vi "Double Array.vi"(8 "Error In":errorcluster) -> (0 "Error Out":errorcluster)   [LabVIEW 2018, in "Tests.lvlib" / "To Msgpack.lvlib"]
uses:
  To Msgpack.lvlib
  <vilib>/addons/_JKI Toolkits/Caraya/classes/Test/Test.lvclass
  src/Toolkit/Toolkit.lvlib
  <vilib>/addons/_JKI Toolkits/Caraya/classes/Assert/Assert.lvclass
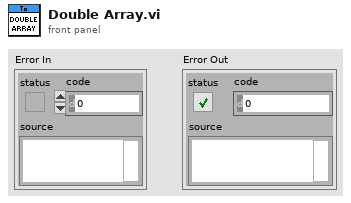
[diagram p1: front panel]
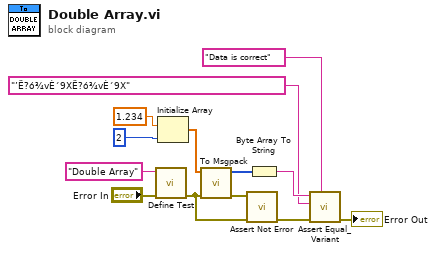
[diagram p0: block diagram]
diagram:
  n1 = call <vilib>:"Define Test.vi"("error in (no error)"="Error In", "Label (VI Title)"="Double Array") -> ("error out"=w9:errorcluster)  [unwired: 9 in]
  n2 = Initialize Array(1.234, 2 ("dimension size")) -> (w7:dbl[])
  n3 = call "To Msgpack.vi"("Error In"=w9, "Anything"=w7) -> ("Error Out"=w10:errorcluster, "Msgpack Data"=w4:u8[])  [unwired: 8 in]
  n4 = call <vilib>:"Assert Not Error.vi"("error in (no error)"=w9, "Not Error?"=w10) -> ("error out"=w11:errorcluster)  [unwired: 9 in]
  n5 = Byte Array To String(unsigned byte array=w4) -> (string=w3:string)
  n6 = call <vilib>:"Assert Equal_Variant.vi"("Label"="Data is correct", "error in (no error)"=w11, "Y"="’Ë?ó¾vÈ´9XË?ó¾vÈ´9X" ("string"), "X"=w3) -> ("error out"=→"Error Out":errorcluster)  [unwired: 7 in]
